vi "Check Limits.vi"(8 "error in (no error)":errorcluster, 11 "System Health Module in":refnum<class "System Health Module.lvclass">) -> (0 "error out":errorcluster, 3 "System Health Module out":refnum<class "System Health Module.lvclass">)   [LabVIEW 2020, in "Volatus.lvlib" / "System Health Module.lvclass"]
uses:
  System Health Module.lvclass
  C:/dev/lv20CE/relink/lv-volatus/Volatus/Module/Module.lvclass
  System Health Module.lvclass/System Health Module.ctl
  Event Level.ctl
  Module/Module.lvclass/Module.ctl
  Module/Module.lvclass
  System SAL/System SAL.lvclass
  Volatus.lvlib
  C:/dev/lv20CE/relink/lv-volatus/Volatus/System Health Module/System Health Module.lvclass
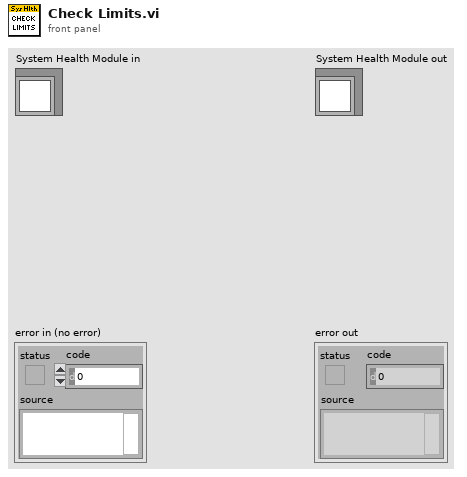
[diagram p1: front panel]
types:
  T1 = typedef "Volatus.lvlib/System Health Module.lvclass/Drive Info.ctl" = cluster{"Config":T2, "Capacity GB":dbl, "Used GB":dbl, "Next Warning":dbl, "Next Error":dbl}
  T2 = typedef "Volatus.lvlib/System Health Module.lvclass/Drive Config.ctl" = cluster{"Path":path, "Warning GB":dbl, "Error GB":dbl}
  T3 = typedef "Volatus.lvlib/Event Level.ctl" = enum16{"Debug", "Info", "Warning", "Error"}
  T4 = typedef "Volatus.lvlib/System SAL.lvclass/Performance Values.ctl" = cluster{"CPU Total %":dbl, "Mem Avail GB":dbl, "Mem Free GB":dbl}
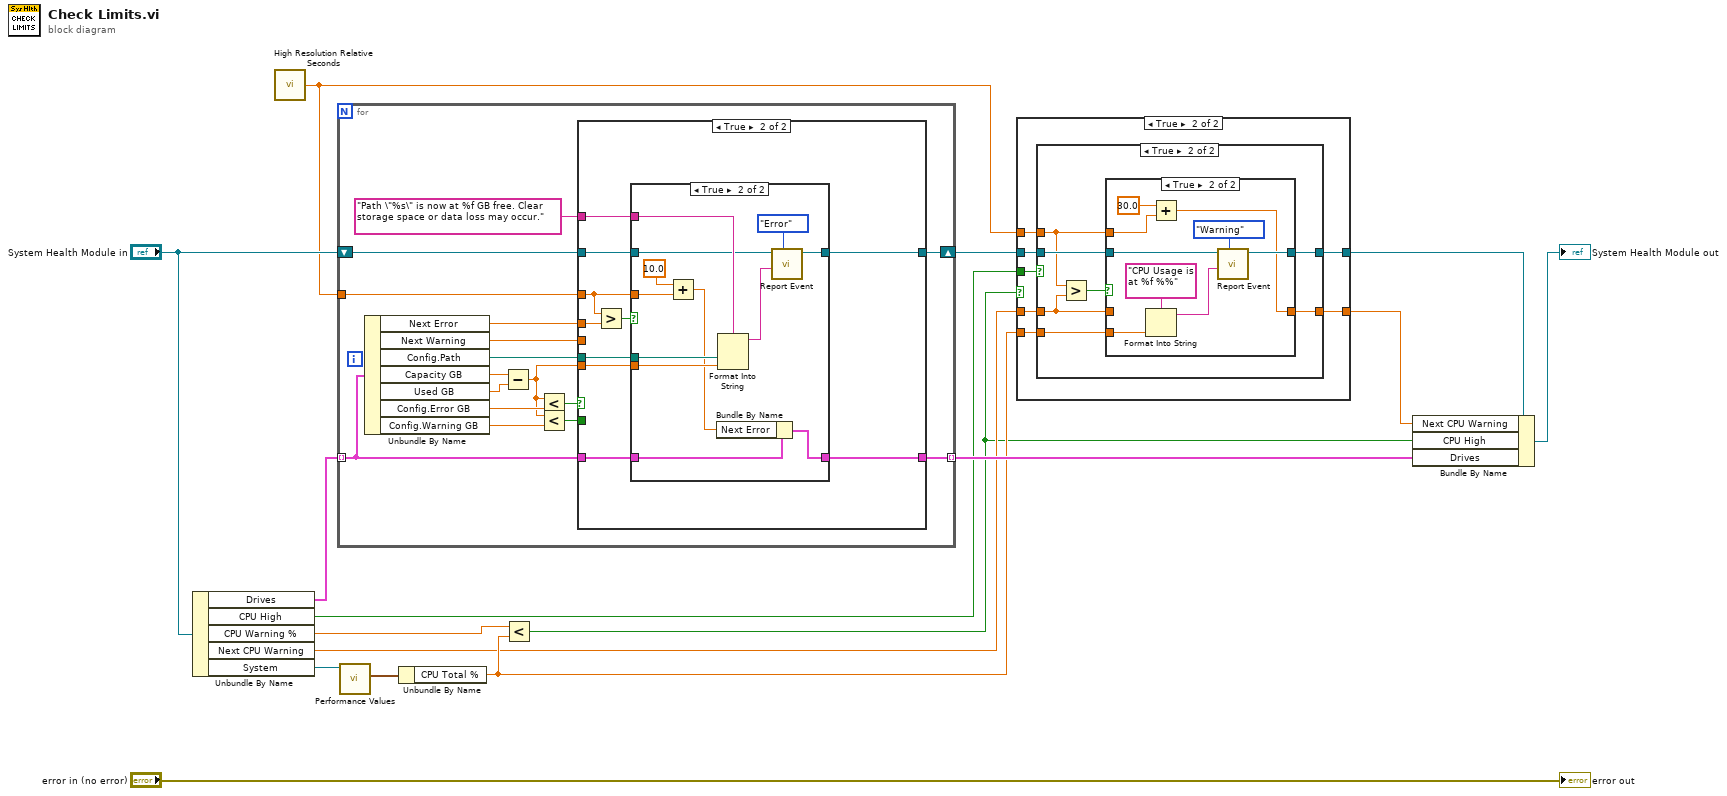
[diagram p0: block diagram]
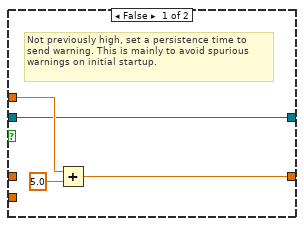
[diagram p3: hidden frame]
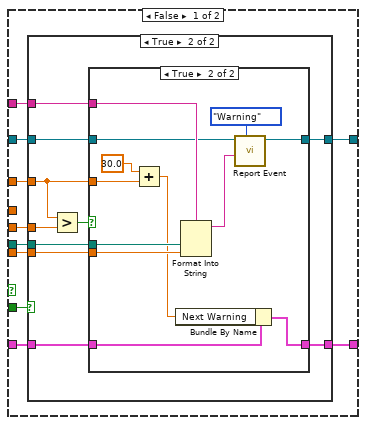
[diagram p5: hidden frame]
diagram:
  n1 = Unbundle By Name("System Health Module in") -> ("Drives"=w15:T1[], "CPU High"=w2:bool, "CPU Warning %"=w9:dbl, "Next CPU Warning"=w5:dbl, "System"=w13:refnum<class "System SAL.lvclass">)
  n2 = call <vilib>:"High Resolution Relative Seconds.vi"() -> ("relative seconds"=w4:dbl)
  n3 = for {
    tunnel: w15 -> [w20] mode=indexing
    shift-right: [w23] -> w8
    shift-left: "System Health Module in" -> [w24]
    tunnel: w4 -> [w21]
    tunnel: [w18] -> w10 mode=indexing
    n4 = Unbundle By Name(w20) -> ("Next Error"=w22:dbl, "Next Warning"=w17:dbl, "Config.Path"=w29:path, "Capacity GB"=w32:dbl, "Used GB"=w31:dbl, "Config.Error GB"=w28:dbl, "Config.Warning GB"=w27:dbl)
    n5 = Subtract(x=w32, y=w31) -> (x-y=w26:dbl)
    n6 = Less?(x=w26, y=w28) -> (x < y?=w30:bool)
    n7 = Less?(x=w26, y=w27) -> (x < y?=w25:bool)
    n8 = case shown="True" w30 {
      tunnel: w29 -> [w40 w77]
      tunnel: "Path \"%s\" is now at %f GB free. Clear storage space or data loss may occur." -> [w39 w78]
      tunnel: w26 -> [w41 w76]
      tunnel: w25 -> [w42 _]
      tunnel: w24 -> [w38 w75]
      tunnel: [w37 w74] -> w23
      tunnel: w22 -> [_ w73]
      tunnel: w21 -> [w36 w71]
      tunnel: w20 -> [w35 w70]
      tunnel: [w34 w69] -> w18
      tunnel: w17 -> [w33 _]
      frame False {
        n9 = case shown="True" w42 {
          tunnel: w41 -> [_ w52]
          tunnel: w40 -> [_ w53]
          tunnel: w39 -> [_ w54]
          tunnel: w38 -> [w44 w51]
          tunnel: [w44 w50] -> w37
          tunnel: w36 -> [_ w46]
          tunnel: w35 -> [w43 w49]
          tunnel: [w43 w48] -> w34
          tunnel: w33 -> [_ w47]
          frame False {
          }
          frame True {
            n10 = Greater?(x=w46, y=w47) -> (0:w45:bool)
            n11 = case shown="True" w45 {
              tunnel: w54 -> [_ w68]
              tunnel: w53 -> [_ w67]
              tunnel: w52 -> [_ w66]
              tunnel: w51 -> [w56 w65]
              tunnel: [w56 w63] -> w50
              tunnel: w46 -> [_ w61]
              tunnel: w49 -> [w55 w59]
              tunnel: [w55 w57] -> w48
              frame False {
              }
              frame True {
                n12 = Add(x=30.0, y=w61) -> (x+y=w58:dbl)
                n13 = Bundle By Name(cluster=w59, "Next Warning"=w58) -> (w57:T1)
                n14 = Format Into String(format string=w68, w67, w66) -> (resulting string=w62:string)  [unwired: 2 in, 1 out]
                n15 = call "Report Event.vi"("Level (Info)"=Event_Level."Warning", "Message"=w62, "Module in"=w65) -> ("Module out"=w63:refnum<class "System Health Module.lvclass">)  [unwired: 7 in, 1 out]
              }
            }
          }
        }
      }
      frame True {
        n16 = Greater?(x=w71, y=w73) -> (0:w72:bool)
        n17 = case shown="True" w72 {
          tunnel: w78 -> [_ w92]
          tunnel: w77 -> [_ w91]
          tunnel: w76 -> [_ w90]
          tunnel: w75 -> [w79 w88]
          tunnel: [w79 w86] -> w74
          tunnel: w71 -> [_ w85]
          tunnel: w70 -> [w80 w83]
          tunnel: [w80 w81] -> w69
          frame False {
          }
          frame True {
            n18 = Add(x=10.0, y=w85) -> (x+y=w82:dbl)
            n19 = Bundle By Name(cluster=w83, "Next Error"=w82) -> (w81:T1)
            n20 = Format Into String(format string=w92, w91, w90) -> (resulting string=w87:string)  [unwired: 2 in, 1 out]
            n21 = call "Report Event.vi"("Level (Info)"=Event_Level."Error", "Message"=w87, "Module in"=w88) -> ("Module out"=w86:refnum<class "System Health Module.lvclass">)  [unwired: 7 in, 1 out]
          }
        }
      }
    }
  }
  n22 = call-dynamic "Performance Values.vi"("System SAL in"=w13) -> ("Performance Values"=w12:T4)  [unwired: 9 in, 1 out]
  n23 = Unbundle By Name(w12) -> ("CPU Total %"=w6:dbl)
  n24 = Less?(x=w9, y=w6) -> (x < y?=w1:bool)
  n25 = case shown="True" w1 {
    tunnel: w8 -> [w93 w101]
    tunnel: [w93 w100] -> w7
    tunnel: w6 -> [_ w99]
    tunnel: w5 -> [w94 w97]
    tunnel: w4 -> [_ w98]
    tunnel: [w94 w96] -> w3
    tunnel: w2 -> [_ w95]
    frame False {
    }
    frame True {
      n26 = case shown="True" w95 {
        tunnel: w101 -> [w102 w112]
        tunnel: [w102 w111] -> w100
        tunnel: w99 -> [_ w110]
        tunnel: w98 -> [w105 w108]
        tunnel: w97 -> [_ w107]
        tunnel: [w103 w106] -> w96
        frame False {
          # "Not previously high, set a persistence time to send warning. This is mainly to avoid spurious warnings on initial startup."
          n27 = Add(x=w105, y=5.0) -> (x+y=w103:dbl)
        }
        frame True {
          n28 = Greater?(x=w108, y=w107) -> (0:w109:bool)
          n29 = case shown="True" w109 {
            tunnel: w112 -> [w113 w122]
            tunnel: [w113 w121] -> w111
            tunnel: w110 -> [_ w118]
            tunnel: w108 -> [_ w120]
            tunnel: w107 -> [w114 _]
            tunnel: [w114 w115] -> w106
            frame False {
            }
            frame True {
              n30 = Format Into String(format string="CPU Usage is at %f %%", w118) -> (resulting string=w116:string)  [unwired: 2 in, 1 out]
              n31 = Add(x=30.0, y=w120) -> (x+y=w115:dbl)
              n32 = call "Report Event.vi"("Level (Info)"=Event_Level."Warning", "Message"=w116, "Module in"=w122) -> ("Module out"=w121:refnum<class "System Health Module.lvclass">)  [unwired: 7 in, 1 out]
            }
          }
        }
      }
    }
  }
  n33 = Bundle By Name(cluster=w7, "Next CPU Warning"=w3, "CPU High"=w1, "Drives"=w10) -> (→"System Health Module out":refnum<class "System Health Module.lvclass">)
  "error out" <- "error in (no error)"
